vi "RT Functions CMA v00.vi"(7 "Function":T5(ring)=enum."V3 Measure", 8 "error in (no error)":errorcluster, 9 "DAQ Trigger":T4={"Trig Source"=0, "Digital Trigger"=FALSE, "Trig Edge"=10171, "Pulse Line"=0, "Pulse On Time"=0} {"Pulse Line" items=["/Line0", "/Line1", "/Line2", "/Line3", "/Line4", "/Line5", "/Line6", "/Line7", "/Line8", "/Line9", "/Line10", "/Line11", "/Line12", "/Line13", "/Line14", "/Line15"]; "Trig Edge" items=["Rising"=10280, "Falling"=10171]; "Trig Source" items=["PFI0", "PFI1", "PFI2", "PFI3", "PFI4", "PFI5", "PFI6", "PFI7", "PFI8", "PFI9", "PFI10", "PFI11", "PFI12", "PFI13", "PFI14", "PFI15"]}, 10 "DAQ Timing":T3={"Number of Samples"=40000, "Samples Per Second"=970000.0, "Sample Mode"=10178, "Timeout (s)"=10.0} {"Sample Mode" items=["Continuous"=10123, "Finite Sample"=10178, "Hardware Timed Single Point"=12522]}, 11 "DAQ Channel":T2={"Channel"=1, "input terminal configuration"=10106, "Input Range Range"=10.0, "Device"="DAQ1"} {"input terminal configuration" items=["default"=-1, "RSE"=10083, "NRSE"=10078, "Differential"=10106, "Pseudodifferential"=12529]; "Input Range Range" items=["+/-10V"=10.0, "+/-5V"=5.0, "+/-2V"=2.0, "+/-1V"=1.0, "+/-0.5V"=0.5, "+/-0.2V"=0.2, "+/-0.1V"=0.1]; "Channel" items=["0"=0, "1"=1, "2"=2, "3"=3, "4"=4, "5"=5, "6"=6, "7"=7, "16"=16, "17"=17, "18"=18, "19"=19, "20"=20, "21"=21, "22"=22, "23"=23]}) -> (0 "error out":errorcluster, 2 "Wfm":waveform(dbl)={"t0"=timestamp(3404415606.9661703 s since 1904-01-01), "dt"=1.0299999999999546e-06, "Y"=array[1600 elements], "attributes"=variant("NI_ChannelName"=variant(string "Voltage"), "NI_UnitDescription"=variant(string "Volts"))}, 3 "Mean":dbl format="%0.2f", 6 "DAQ Pusle":T1)   [LabVIEW 2013]
uses:
  <vilib>/Analysis/baseanly.llb/Mean (DBL).vi
  <vilib>/Waveform/WDTOps.llb/WDT Get Waveform Subset DBL.vi
  <vilib>/Analysis/NI_AALBase.lvlib
panel:
  out "V2_Wfm 3":waveform(dbl)
  out "V1_Wfm 2":waveform(dbl)
  out "V2_Wfm 2":waveform(dbl)
  out "V3_Wfm":waveform(dbl)
  out "V2_Wfm":waveform(dbl)
  out "V1_Wfm":waveform(dbl)
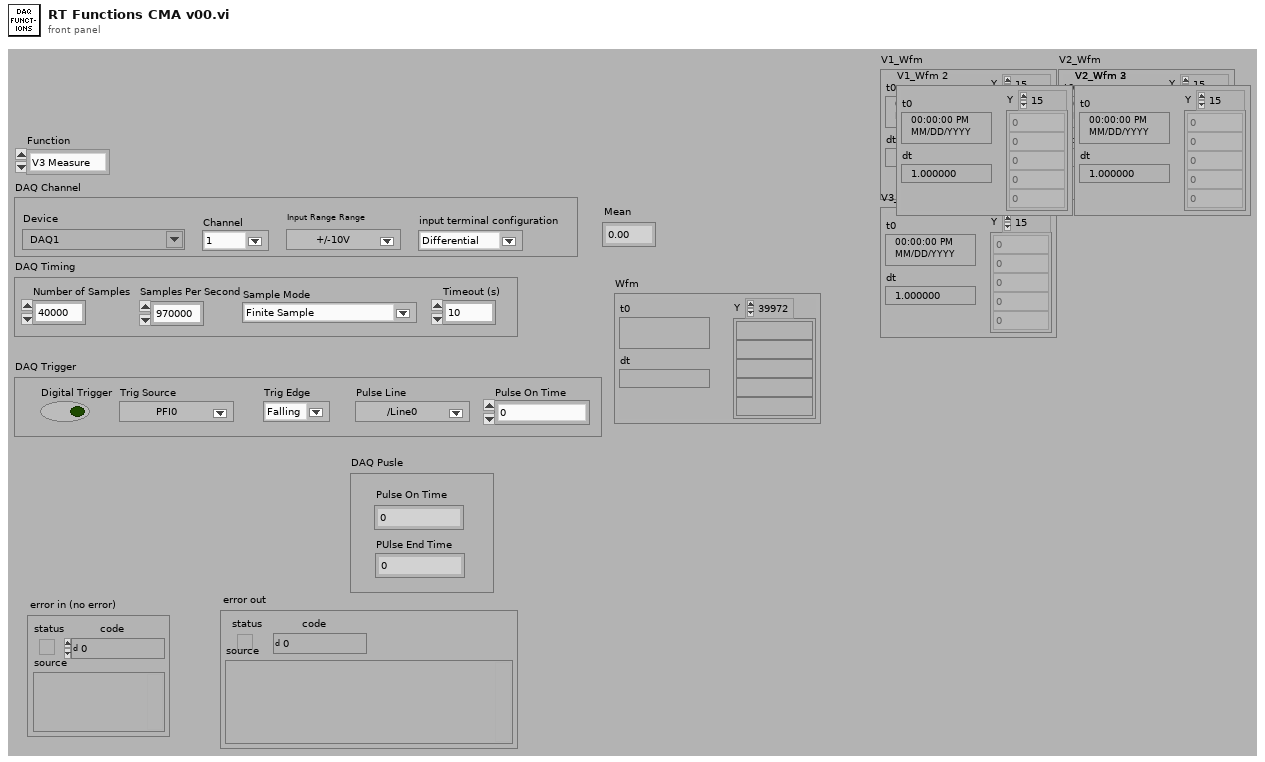
[diagram p1: front panel]
types:
  T1 = cluster{"Pulse On Time":u32, "PUlse End Time":u32}
  T2 = cluster{"Channel":u16, "input terminal configuration":i32, "Input Range Range":dbl, "Device":string}
  T3 = cluster{"Number of Samples":u32, "Samples Per Second":dbl, "Sample Mode":i32, "Timeout (s)":dbl}
  T4 = cluster{"Trig Source":u16, "Digital Trigger":bool, "Trig Edge":i32, "Pulse Line":u16, "Pulse On Time":u32}
  T5 = enum32{"V1 Measure", "V2 Measure", "V2a Measure", "V3 Measure", "CS_Measure", "TS_Measure", "Pulse On", "Pulse Off"}
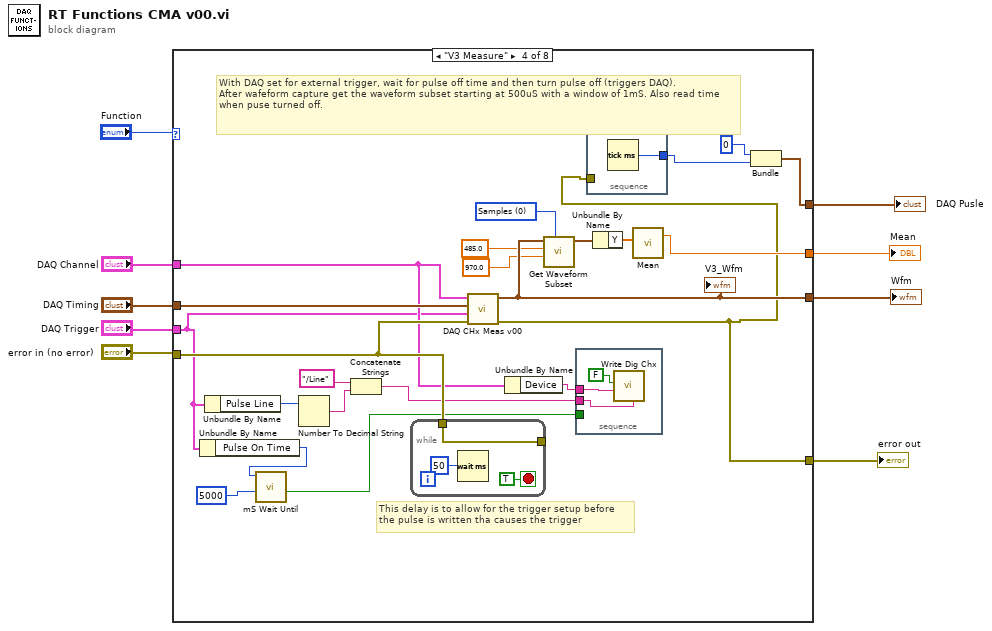
[diagram p0: block diagram]
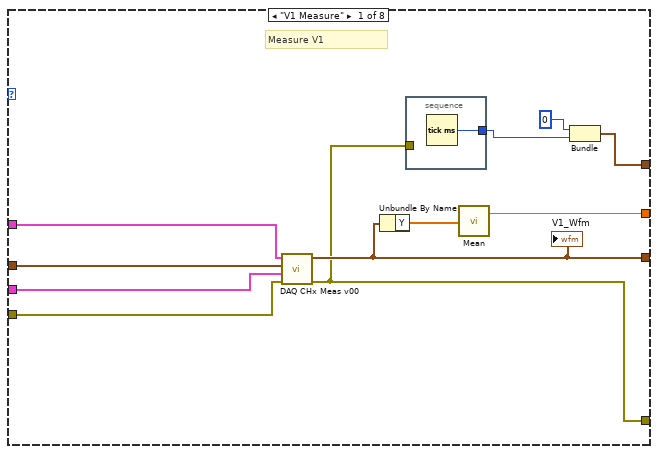
[diagram p2: hidden frame]
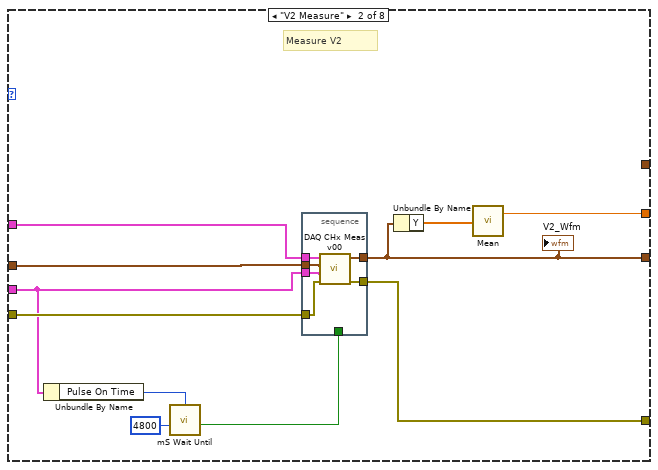
[diagram p3: hidden frame]
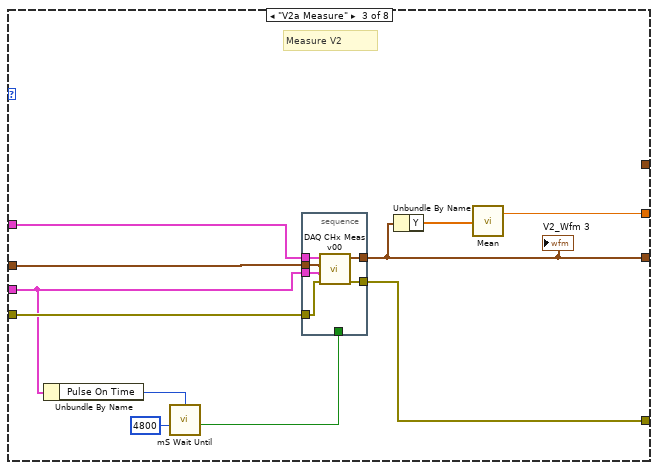
[diagram p4: hidden frame]
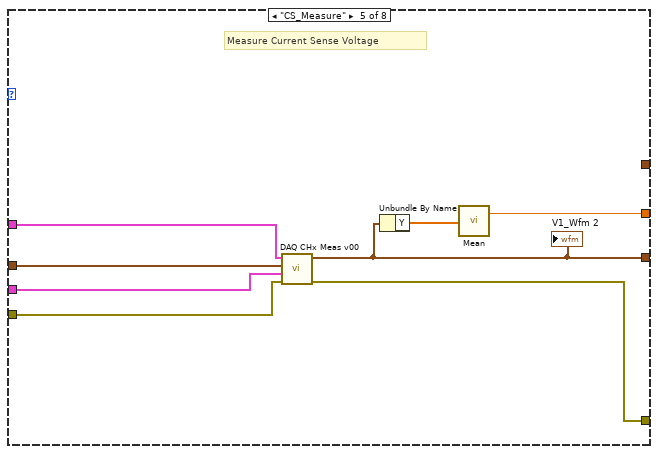
[diagram p5: hidden frame]
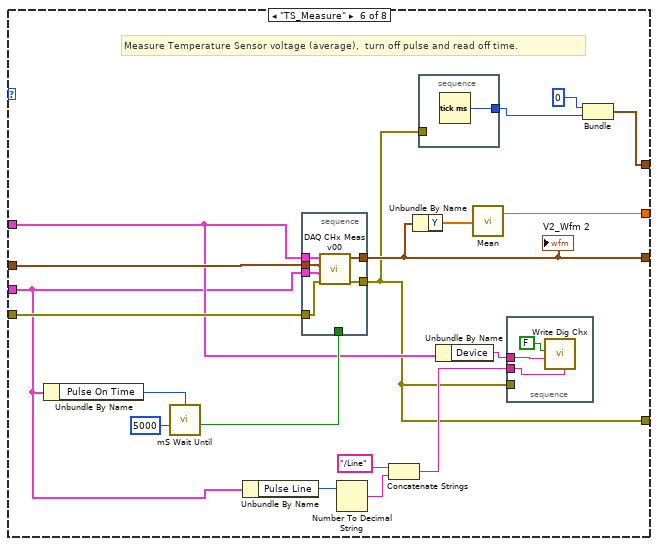
[diagram p6: hidden frame]
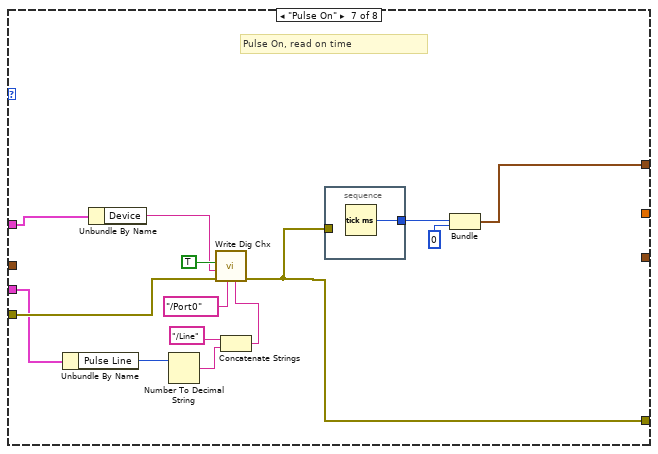
[diagram p7: hidden frame]
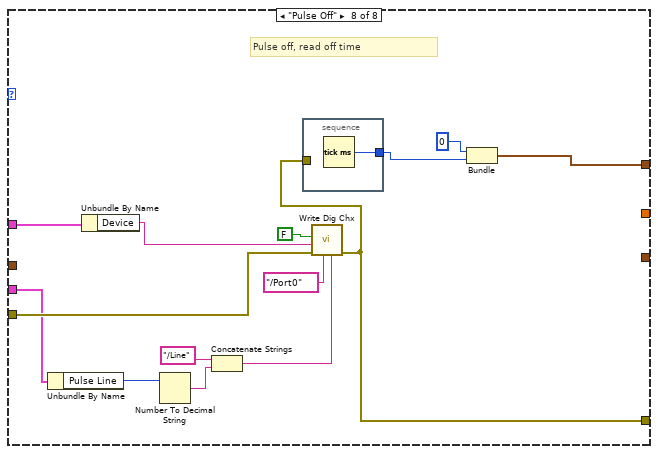
[diagram p8: hidden frame]
diagram:
  n1 = case shown="\"V3 Measure\"" "Function" {
    tunnel: "error in (no error)" -> [w20 w31 w48 w75 w93 w112 w135 w150]
    tunnel: [w10 w32 w49 w56 w92 w94 w131 w146] -> w8
    tunnel: "DAQ Channel" -> [w14 w26 w43 w74 w86 w103 w134 w149]
    tunnel: "DAQ Timing" -> [w19 w30 w47 w78 w91 w111 _ _]
    tunnel: "DAQ Trigger" -> [w18 w22 w39 w60 w90 w99 w126 w141]
    tunnel: [w17 w28 w45 w72 w89 w109 _ _] -> w3
    tunnel: [w15 w27 w44 w76 w87 w108 _ _] -> w2
    tunnel: [w11 _ _ w57 _ w95 w123 w140] -> w1
    frame "V1 Measure" {
      # "Measure V1"
      n2 = call "DAQ CHx Meas v00.vi"("error in"=w20, "DAQ Trigger"=w18, "DAQ Timing"=w19, "DAQ Channel"=w14) -> ("error out"=w10:errorcluster, "Waveform"=w17:waveform(dbl))  [unwired: 6 in]
      "V1_Wfm" <- w17
      n3 = Unbundle By Name(w17) -> ("Y"=w16:dbl[])
      n4 = stacked-sequence {
        tunnel: [w21] -> w13
        tunnel: w10 -> [_]
        frame #0 {
          n5 = Tick Count (ms)() -> (millisecond timer value=w21:u32)
        }
      }
      n6 = call-poly <vilib>:"Mean.vi"("X"=w16) -> ("mean"=w15:dbl)  [unwired: 1 out]
      n7 = Bundle(u32 0, "millisecond timer value"=w13) -> (w11:cluster{u32, "millisecond timer value":u32})  [unwired: 1 in]
    }
    frame "V2 Measure" {
      # "Measure V2"
      n8 = Unbundle By Name(w22) -> ("Pulse On Time"=w23:u32)
      n9 = call "mS Wait Until.vi"("mS Delta"=u16 4800, "mS Start Time"=w23) -> ("Done"=w24:bool)  [unwired: 8 in, 1 out]
      n10 = stacked-sequence {
        tunnel: [w38] -> w32
        tunnel: w31 -> [w37]
        tunnel: w30 -> [w36]
        tunnel: w22 -> [w35]
        tunnel: [w34] -> w28
        tunnel: w26 -> [w33]
        tunnel: w24 -> [_]
        frame #0 {
          n11 = call "DAQ CHx Meas v00.vi"("error in"=w37, "DAQ Trigger"=w35, "DAQ Timing"=w36, "DAQ Channel"=w33) -> ("error out"=w38:errorcluster, "Waveform"=w34:waveform(dbl))  [unwired: 6 in]
        }
      }
      "V2_Wfm" <- w28
      n12 = Unbundle By Name(w28) -> ("Y"=w29:dbl[])
      n13 = call-poly <vilib>:"Mean.vi"("X"=w29) -> ("mean"=w27:dbl)  [unwired: 1 out]
    }
    frame "V2a Measure" {
      # "Measure V2"
      n14 = Unbundle By Name(w39) -> ("Pulse On Time"=w40:u32)
      n15 = call "mS Wait Until.vi"("mS Delta"=u16 4800, "mS Start Time"=w40) -> ("Done"=w41:bool)  [unwired: 8 in, 1 out]
      n16 = stacked-sequence {
        tunnel: [w55] -> w49
        tunnel: w48 -> [w54]
        tunnel: w47 -> [w53]
        tunnel: w39 -> [w52]
        tunnel: [w51] -> w45
        tunnel: w43 -> [w50]
        tunnel: w41 -> [_]
        frame #0 {
          n17 = call "DAQ CHx Meas v00.vi"("error in"=w54, "DAQ Trigger"=w52, "DAQ Timing"=w53, "DAQ Channel"=w50) -> ("error out"=w55:errorcluster, "Waveform"=w51:waveform(dbl))  [unwired: 6 in]
        }
      }
      "V2_Wfm 3" <- w45
      n18 = Unbundle By Name(w45) -> ("Y"=w46:dbl[])
      n19 = call-poly <vilib>:"Mean.vi"("X"=w46) -> ("mean"=w44:dbl)  [unwired: 1 out]
    }
    frame "V3 Measure" {
      w71 = u16 0 items=["Samples", "Relative Time"] ("start/duration format")
      # "With DAQ set for external trigger, wait for pulse off time and then turn pulse off (triggers DAQ).\nAfter wafeform capture get the waveform subset starting at 500uS with a window of 1mS. Also read time when puse turned off."
      # "This delay is to allow for the trigger setup before\nthe pulse is written tha causes the trigger"
      n20 = Unbundle By Name(w60) -> ("Pulse On Time"=w65:u32)
      n21 = Unbundle By Name(w60) -> ("Pulse Line"=w64:u16)
      n22 = call "mS Wait Until.vi"("mS Delta"=u16 5000, "mS Start Time"=w65) -> ("Done"=w66:bool)  [unwired: 8 in, 1 out]
      n23 = Number To Decimal String(number=w64) -> (decimal integer string=w63:string)  [unwired: 1 in]
      n24 = Concatenate Strings("/Line", w63) -> (w61:string)
      n25 = while {
        tunnel: w75 -> [w83]
        tunnel: [w83] -> _
        stop <- TRUE stop-if-true
        n26 = Wait (ms)(milliseconds to wait=u32 50) -> ()  [unwired: 1 out]
      }
      n27 = call "DAQ CHx Meas v00.vi"("error in"=w75, "DAQ Trigger"=w60, "DAQ Timing"=w78, "DAQ Channel"=w74) -> ("error out"=w56:errorcluster, "Waveform"=w72:waveform(dbl))  [unwired: 6 in]
      "V3_Wfm" <- w72
      n28 = Unbundle By Name(w74) -> ("Device"=w73:string)
      n29 = call-poly <vilib>:"Get Waveform Subset.vi"("start/duration format"=w71, "duration"=970.0, "start samples/time"=485.0, "waveform in"=w72) -> ("waveform out"=w68:waveform(dbl))  [unwired: 2 in, 3 out]
      n30 = stacked-sequence {
        tunnel: w73 -> [w81]
        tunnel: w61 -> [w80]
        tunnel: w66 -> [_]
        frame #0 {
          n31 = call "Write Dig Chx.vi"("Line"=w80, "Device"=w81, "Ch Value"=FALSE) -> ()  [unwired: 8 in, 1 out]
        }
      }
      n32 = stacked-sequence {
        tunnel: [w79] -> w58
        tunnel: w56 -> [_]
        frame #0 {
          n33 = Tick Count (ms)() -> (millisecond timer value=w79:u32)
        }
      }
      n34 = Unbundle By Name(w68) -> ("Y"=w77:dbl[])
      n35 = call-poly <vilib>:"Mean.vi"("X"=w77) -> ("mean"=w76:dbl)  [unwired: 1 out]
      n36 = Bundle(u32 0, "millisecond timer value"=w58) -> (w57:cluster{u32, "millisecond timer value":u32})  [unwired: 1 in]
    }
    frame "CS_Measure" {
      # "Measure Current Sense Voltage"
      n37 = call "DAQ CHx Meas v00.vi"("error in"=w93, "DAQ Trigger"=w90, "DAQ Timing"=w91, "DAQ Channel"=w86) -> ("error out"=w92:errorcluster, "Waveform"=w89:waveform(dbl))  [unwired: 6 in]
      "V1_Wfm 2" <- w89
      n38 = Unbundle By Name(w89) -> ("Y"=w88:dbl[])
      n39 = call-poly <vilib>:"Mean.vi"("X"=w88) -> ("mean"=w87:dbl)  [unwired: 1 out]
    }
    frame "TS_Measure" {
      # "Measure Temperature Sensor voltage (average),  turn off pulse and read off time."
      n40 = Unbundle By Name(w99) -> ("Pulse On Time"=w105:u32)
      n41 = call "mS Wait Until.vi"("mS Delta"=u16 5000, "mS Start Time"=w105) -> ("Done"=w106:bool)  [unwired: 8 in, 1 out]
      n42 = Unbundle By Name(w99) -> ("Pulse Line"=w100:u16)
      n43 = stacked-sequence {
        tunnel: [w122] -> w94
        tunnel: w112 -> [w121]
        tunnel: w111 -> [w120]
        tunnel: w99 -> [w119]
        tunnel: [w118] -> w109
        tunnel: w103 -> [w117]
        tunnel: w106 -> [_]
        frame #0 {
          n44 = call "DAQ CHx Meas v00.vi"("error in"=w121, "DAQ Trigger"=w119, "DAQ Timing"=w120, "DAQ Channel"=w117) -> ("error out"=w122:errorcluster, "Waveform"=w118:waveform(dbl))  [unwired: 6 in]
        }
      }
      "V2_Wfm 2" <- w109
      n45 = Number To Decimal String(number=w100) -> (decimal integer string=w101:string)  [unwired: 1 in]
      n46 = Concatenate Strings("/Line", w101) -> (w98:string)
      n47 = Unbundle By Name(w109) -> ("Y"=w110:dbl[])
      n48 = stacked-sequence {
        tunnel: [w113] -> w97
        tunnel: w94 -> [_]
        frame #0 {
          n49 = Tick Count (ms)() -> (millisecond timer value=w113:u32)
        }
      }
      n50 = Unbundle By Name(w103) -> ("Device"=w104:string)
      n51 = call-poly <vilib>:"Mean.vi"("X"=w110) -> ("mean"=w108:dbl)  [unwired: 1 out]
      n52 = stacked-sequence {
        tunnel: w104 -> [w115]
        tunnel: w98 -> [w114]
        tunnel: w94 -> [_]
        frame #0 {
          n53 = call "Write Dig Chx.vi"("Line"=w114, "Device"=w115, "Ch Value"=FALSE) -> ()  [unwired: 8 in, 1 out]
        }
      }
      n54 = Bundle(u32 0, "millisecond timer value"=w97) -> (w95:cluster{u32, "millisecond timer value":u32})  [unwired: 1 in]
    }
    frame "Pulse On" {
      # "Pulse On, read on time"
      n55 = Unbundle By Name(w126) -> ("Pulse Line"=w128:u16)
      n56 = Unbundle By Name(w134) -> ("Device"=w133:string)
      n57 = Number To Decimal String(number=w128) -> (decimal integer string=w129:string)  [unwired: 1 in]
      n58 = Concatenate Strings("/Line", w129) -> (w127:string)
      n59 = call "Write Dig Chx.vi"("Line"=w127, "Port"="/Port0", "error in"=w135, "Device"=w133, "Ch Value"=TRUE) -> ("error out"=w131:errorcluster)  [unwired: 6 in]
      n60 = stacked-sequence {
        tunnel: w131 -> [_]
        tunnel: [w137] -> w125
        frame #0 {
          n61 = Tick Count (ms)() -> (millisecond timer value=w137:u32)
        }
      }
      n62 = Bundle("millisecond timer value"=w125, u32 0) -> (w123:cluster{"millisecond timer value":u32, u32})  [unwired: 1 in]
    }
    frame "Pulse Off" {
      # "Pulse off, read off time"
      n63 = Unbundle By Name(w141) -> ("Pulse Line"=w143:u16)
      n64 = Unbundle By Name(w149) -> ("Device"=w148:string)
      n65 = Number To Decimal String(number=w143) -> (decimal integer string=w144:string)  [unwired: 1 in]
      n66 = Concatenate Strings("/Line", w144) -> (w142:string)
      n67 = call "Write Dig Chx.vi"("Line"=w142, "Port"="/Port0", "error in"=w150, "Device"=w148, "Ch Value"=FALSE) -> ("error out"=w146:errorcluster)  [unwired: 6 in]
      n68 = stacked-sequence {
        tunnel: w146 -> [_]
        tunnel: [w152] -> w139
        frame #0 {
          n69 = Tick Count (ms)() -> (millisecond timer value=w152:u32)
        }
      }
      n70 = Bundle(u32 0, "millisecond timer value"=w139) -> (w140:cluster{u32, "millisecond timer value":u32})  [unwired: 1 in]
    }
  }
  "error out" <- w8
  "Wfm" <- w3
  "Mean" <- w2
  "DAQ Pusle" <- w1
